vi "CSE routine - Access to Context Error Record.vi"(7 "cmd (0: read)":i32(ring) items=["read", "write", "reset"], 8 "error message in":string, 9 "error code in":i32, 10 "Stm Index in":i32=-1, 11 "CSE RefNum":T1) -> (0 "error message out":string, 1 "error code out":i32, 2 "Stm Index out":i32=-1, 3 "dup CSE RefNum":T1, 4 "execStatus":i32)   [LabVIEW 2021]
doc: "::: CalcExpress Toolkit :::\nCopyright (c) 2000-2026 Konstantin Shifershteyn. All rights reserved."
uses:
  CSE Instance RefNum.ctl
  cersrc/celveng32.dll
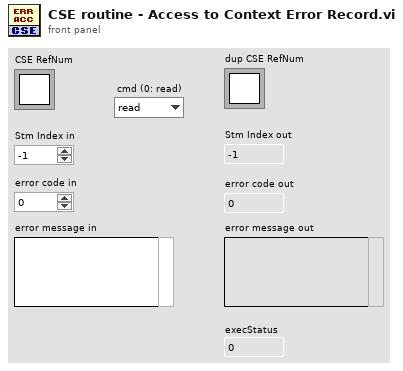
[diagram p1: front panel]
types:
  T1 = typedef "CSE Instance RefNum.ctl" = refnum<k1>
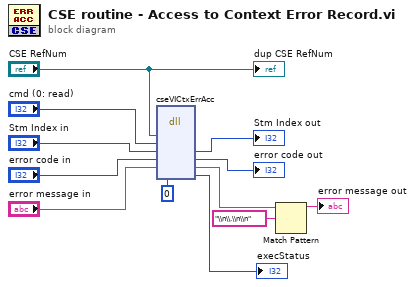
[diagram p0: block diagram]
diagram:
  n1 = dll-call lib="C:/LV Projects/CalcExpress 40 LV2021/vi.lib/addons/CalcExpress/cersrc/celveng*.dll" fn="cseVICtxErrAcc"("instRef"="CSE RefNum", "cmd"="cmd (0: read)", "StmIndex"="Stm Index in", "ErrCode"="error code in", "ErrMsg"="error message in", "execStat"=0) -> ("StmIndex"=→"Stm Index out":i32, "ErrCode"=→"error code out":i32, "ErrMsg"=w2:string, "execStat"=→"execStatus":i32)  [unwired: 6 in, 2 out]
  n2 = Match Pattern(string=w2, regular expression="\\n\\.\\n\\n") -> (before substring=→"error message out":string)  [unwired: 1 in, 3 out]
  "dup CSE RefNum" <- "CSE RefNum"
